vi "AI_Get_Candidates.vi"(0 "Grid":enum8{"Empty", "Black", "White"}[][](array[ring])=[[enum."Empty", enum."Empty", enum."Empty", enum."Empty", enum."Empty", enum."Empty", enum."Empty", enum."Empty", enum."Empty", enum."Empty", enum."Empty", enum."Empty", enum."Empty", enum."Empty", enum."Empty"], [enum."Empty", enum."Empty", enum."Empty", enum."Empty", enum."Empty", enum."Empty", enum."Empty", enum."Empty", enum."Empty", enum."Empty", enum."Empty", enum."Empty", enum."Empty", enum."Empty", enum."Empty"], [enum."Empty", enum."Empty", enum."Empty", enum."Empty", enum."Empty", enum."Empty", enum."Empty", enum."Empty", enum."Empty", enum."Empty", enum."Empty", enum."Empty", enum."Empty", enum."Empty", enum."Empty"], [enum."Empty", enum."Empty", enum."Empty", enum."Empty", enum."Empty", enum."Empty", enum."Empty", enum."Empty", enum."Empty", enum."Empty", enum."Empty", enum."Empty", enum."Empty", enum."Empty", enum."Empty"], [enum."Empty", enum."Empty", enum."Empty", enum."Empty", enum."Empty", enum."Empty", enum."Empty", enum."Empty", enum."Empty", enum."Empty", enum."Empty", enum."Empty", enum."Empty", enum."Empty", enum."Empty"], [enum."Empty", enum."Empty", enum."Empty", enum."Empty", enum."Empty", enum."Empty", enum."Empty", enum."Empty", enum."Empty", enum."Empty", enum."Empty", enum."Empty", enum."Empty", enum."Empty", enum."Empty"], [enum."Empty", enum."Empty", enum."Empty", enum."Empty", enum."Empty", enum."Empty", enum."Empty", enum."Empty", enum."Empty", enum."Empty", enum."Empty", enum."Empty", enum."Empty", enum."Empty", enum."Empty"], [enum."Empty", enum."Empty", enum."Empty", enum."Empty", enum."Empty", enum."Empty", enum."Empty", enum."Empty", enum."Empty", enum."Empty", enum."Empty", enum."Empty", enum."Empty", enum."Empty", enum."Empty"], [enum."Empty", enum."Empty", enum."Empty", enum."Empty", enum."Empty", enum."Empty", enum."Empty", enum."Empty", enum."Empty", enum."Empty", enum."Empty", enum."Empty", enum."Empty", enum."Empty", enum."Empty"], [enum."Empty", enum."Empty", enum."Empty", enum."Empty", enum."Empty", enum."Empty", enum."Empty", enum."Empty", enum."Empty", enum."Empty", enum."Empty", enum."Empty", enum."Empty", enum."Empty", enum."Empty"], [enum."Empty", enum."Empty", enum."Empty", enum."Empty", enum."Empty", enum."Empty", enum."Empty", enum."Empty", enum."Empty", enum."Empty", enum."Empty", enum."Empty", enum."Empty", enum."Empty", enum."Empty"], [enum."Empty", enum."Empty", enum."Empty", enum."Empty", enum."Empty", enum."Empty", enum."Empty", enum."Empty", enum."Empty", enum."Empty", enum."Empty", enum."Empty", enum."Empty", enum."Empty", enum."Empty"], [enum."Empty", enum."Empty", enum."Empty", enum."Empty", enum."Empty", enum."Empty", enum."Empty", enum."Empty", enum."Empty", enum."Empty", enum."Empty", enum."Empty", enum."Empty", enum."Empty", enum."Empty"], [enum."Empty", enum."Empty", enum."Empty", enum."Empty", enum."Empty", enum."Empty", enum."Empty", enum."Empty", enum."Empty", enum."Empty", enum."Empty", enum."Empty", enum."Empty", enum."Empty", enum."Empty"], [enum."Empty", enum."Empty", enum."Empty", enum."Empty", enum."Empty", enum."Empty", enum."Empty", enum."Empty", enum."Empty", enum."Empty", enum."Empty", enum."Empty", enum."Empty", enum."Empty", enum."Empty"]], 11 "error in":errorcluster) -> (4 "Rows":i32[](array[numeric]), 6 "Cols":i32[](array[numeric]), 8 "Count":i32, 15 "error out":errorcluster)   [LabVIEW 2026]
doc: "후보 수 생성: 빈 칸 중 반경 2(5x5) 안에 돌이 하나라도 있는 칸. 빈 보드면 (7,7) 하나."
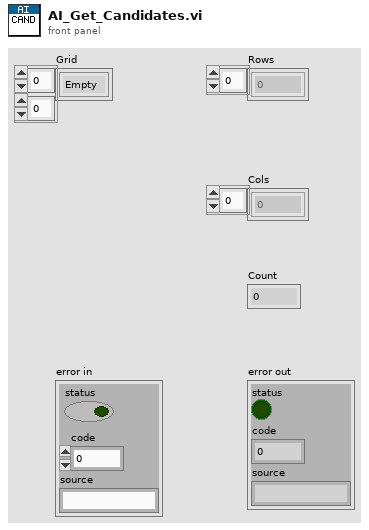
[diagram p1: front panel]
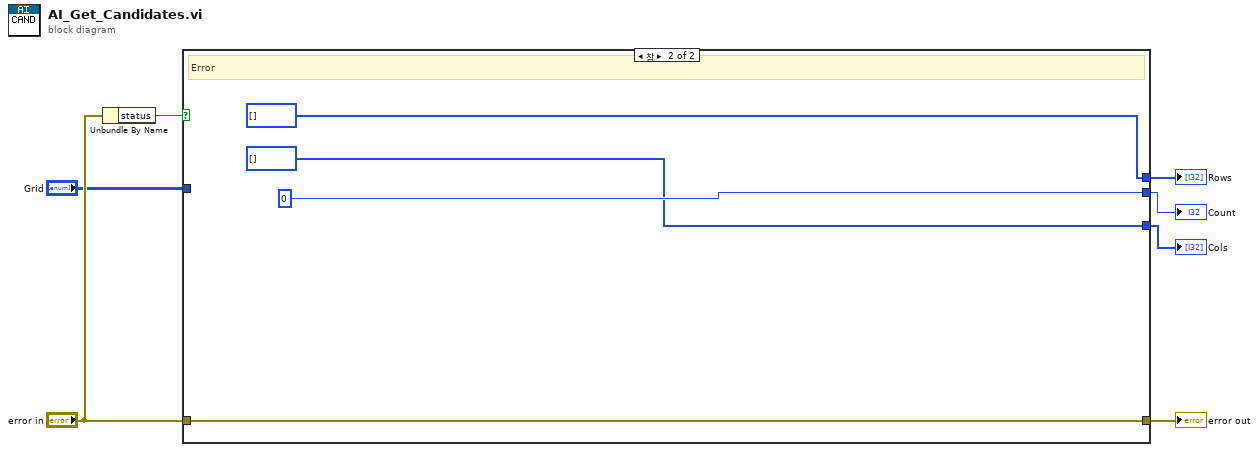
[diagram p0: block diagram]
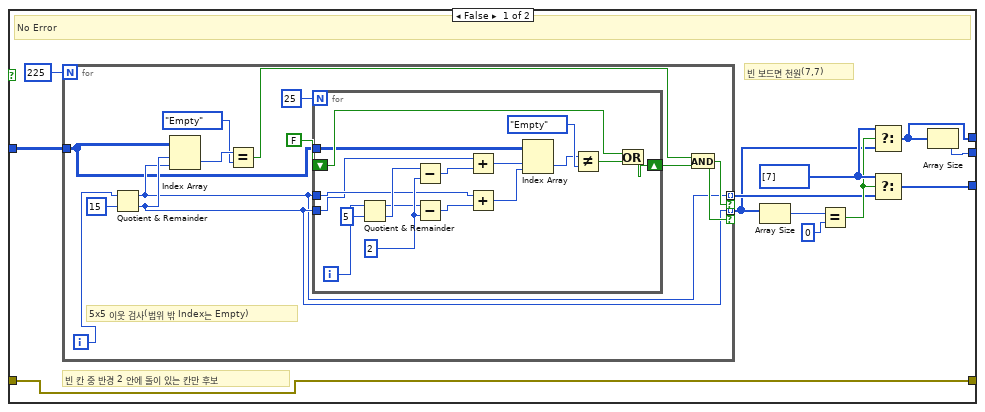
[diagram p2: hidden frame]
diagram:
  n1 = Unbundle By Name("error in") -> ("status"=w3:bool)
  n2 = case shown="참" w3 {
    tunnel: "Grid" -> [w8 _]
    tunnel: "error in" -> [w9 w49]
    tunnel: [w9 w49] -> w7
    tunnel: [w17 i32[] []] -> w4
    tunnel: [w18 i32[] []] -> w5
    tunnel: [w19 0] -> w6
    frame False {
      w16 = i32[] [7]
      # "빈 보드면 천원(7,7)"
      # "빈 칸 중 반경 2 안에 돌이 있는 칸만 후보"
      # "No Error"
      n3 = for {
        N: 225 -> [_]
        tunnel: w8 -> [w21]
        tunnel: [w24] -> w11 mode=indexing if=w31
        tunnel: [w23] -> w12 mode=indexing if=w31
        i -> [w20]
        # "5x5 이웃 검사(범위 밖 Index는 Empty)"
        n4 = Quotient & Remainder(x=w20, y=15) -> (x-y*floor(x/y)=w23:i32, floor(x/y)=w24:i32)
        n5 = Index Array(array=w21, index (row)=w24, index (col)=w23) -> (element=w26:enum8{"Empty", "Black", "White"})
        n6 = Equal?(x=w26, y=enum8{"Empty", "Black", "White"}."Empty") -> (x = y?=w27:bool)
        n7 = for {
          N: 25 -> [_]
          shift-right: [w47] -> w30
          shift-left: FALSE -> [w48]
          tunnel: w24 -> [w34]
          tunnel: w23 -> [w35]
          tunnel: w21 -> [w33]
          i -> [w32]
          w39 = 2
          n8 = Quotient & Remainder(x=w32, y=5) -> (x-y*floor(x/y)=w37:i32, floor(x/y)=w38:i32)
          n9 = Subtract(x=w38, y=w39) -> (x-y=w40:i32)
          n10 = Subtract(x=w37, y=w39) -> (x-y=w42:i32)
          n11 = Add(x=w34, y=w40) -> (x+y=w41:i32)
          n12 = Add(x=w35, y=w42) -> (x+y=w43:i32)
          n13 = Index Array(array=w33, index (row)=w41, index (col)=w43) -> (element=w44:enum8{"Empty", "Black", "White"})
          n14 = Not Equal?(x=w44, y=enum8{"Empty", "Black", "White"}."Empty") -> (x != y?=w46:bool)
          n15 = Or(x=w48, y=w46) -> (x .or. y?=w47:bool)
        }
        n16 = And(x=w27, y=w30) -> (x .and. y?=w31:bool)
      }
      n17 = Array Size(array=w11) -> (size(s)=w13:i32)
      n18 = Equal?(x=w13, y=0) -> (x = y?=w15:bool)
      n19 = Select(t=w16, s=w15, f=w11) -> (s? t:f=w17:i32[])
      n20 = Select(t=w16, s=w15, f=w12) -> (s? t:f=w18:i32[])
      n21 = Array Size(array=w17) -> (size(s)=w19:i32)
    }
    frame True {
      # "Error"
    }
  }
  "Rows" <- w4
  "Cols" <- w5
  "Count" <- w6
  "error out" <- w7
